vi "FindTemplateMethod.vi"(10 "TemplatePath To Use first":path, 11 "TemplatePath in":path) -> (3 "TemplatePath out":path)   [LabVIEW 2020, in "ClassWriterNative.lvclass"]
uses:
  ClassWriterNative.lvclass
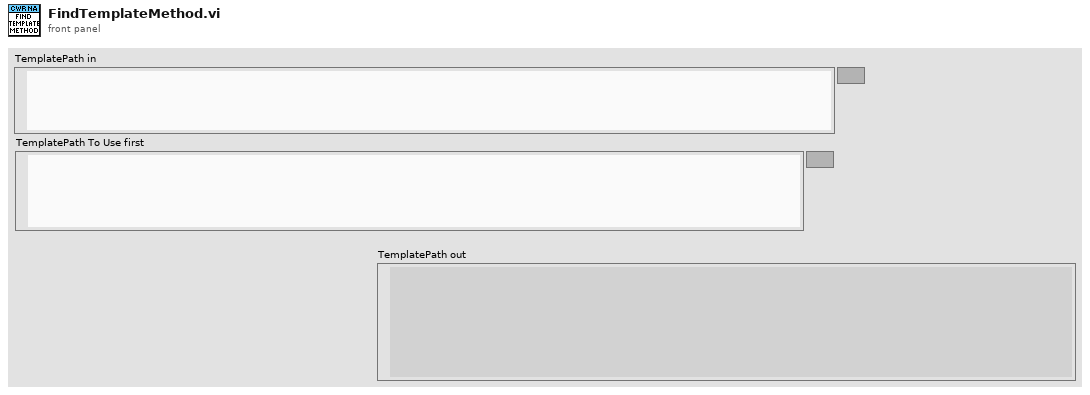
[diagram p1: front panel]
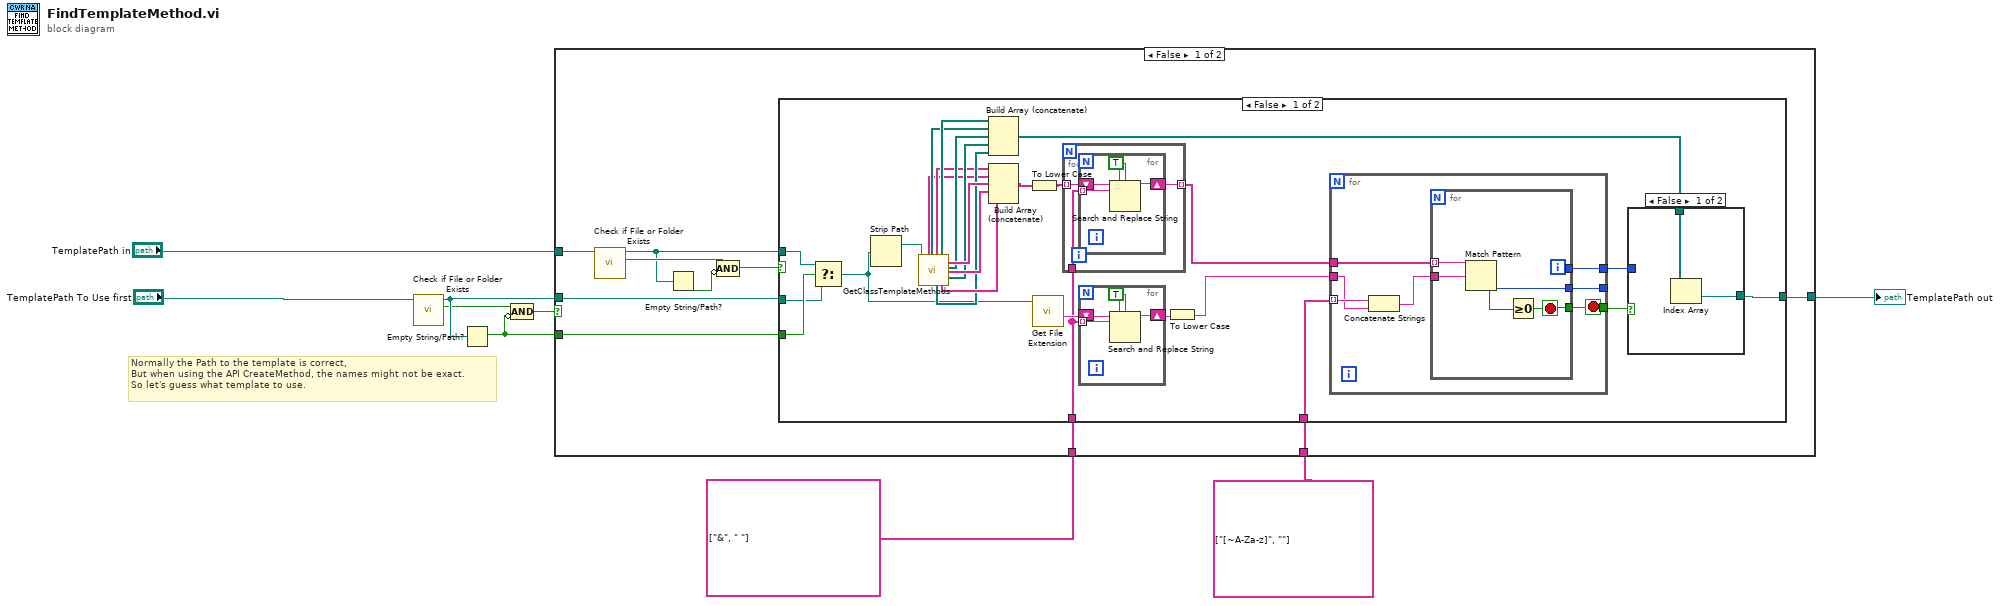
[diagram p0: block diagram]
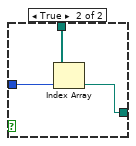
[diagram p2: hidden frame]
diagram:
  # "Normally the Path to the template is correct, \nBut when using the API CreateMethod, the names might not be exact.\nSo let's guess what template to use."
  n1 = call <vilib>:"Check if File or Folder Exists.vi"("path"="TemplatePath To Use first") -> ("file or folder exists?"=w5:bool, "dup path"=w6:path)  [unwired: 8 in, 1 out]
  n2 = Empty String/Path?(string/path=w6) -> (empty?=w1:bool)
  n3 = Compound Arithmetic op=AND(w5, invert w1) -> (w4:bool)
  n4 = case shown="False" w4 {
    tunnel: [w15 w76] -> w8
    tunnel: w6 -> [w12 w76]
    tunnel: "TemplatePath in" -> [w19 _]
    tunnel: string[] ["&", " "] -> [w14 _]
    tunnel: string[] ["[~A-Za-z]", ""] -> [w13 _]
    tunnel: w1 -> [w10 _]
    frame False {
      n5 = call <vilib>:"Check if File or Folder Exists.vi"("path"=w19) -> ("file or folder exists?"=w17:bool, "dup path"=w11:path)  [unwired: 8 in, 1 out]
      n6 = Empty String/Path?(string/path=w11) -> (empty?=w18:bool)
      n7 = Compound Arithmetic op=AND(w17, invert w18) -> (w16:bool)
      n8 = case shown="False" w16 {
        tunnel: w12 -> [w26 _]
        tunnel: [w30 w75] -> w15
        tunnel: w14 -> [w32 _]
        tunnel: w13 -> [w43 _]
        tunnel: w11 -> [w25 w75]
        tunnel: w10 -> [w27 _]
        frame False {
          n9 = Select(t=w25, s=w27, f=w26) -> (s? t:f=w24:path)
          n10 = Strip Path(path=w24) -> (stripped path=w28:path)  [unwired: 1 out]
          n11 = call "GetClassTemplateMethods.vi"("MethodTemplatePath"=w28) -> ("InterfaceMethodNames"=w20:string[], "InterfaceMethodPaths"=w22:path[], "NormalMethodNames"=w21:string[], "PropertyNodeMethodPaths"=w37:path[], "NormalMethodPaths"=w23:path[], "PropertyNodeMethodNames"=w40:string[], "OverrideMethodNames"=w42:string[], "OverrideMethodPaths"=w39:path[], "PropertyMethodNames"=w41:string[], "PropertyMethodPaths"=w38:path[])  [unwired: 8 in, 1 out]
          n12 = Build Array (concatenate)(w23, w22, w39, w38, w37) -> (w34:path[])
          n13 = Build Array (concatenate)(w21, w20, w42, w41, w40) -> (w36:string[])
          n14 = To Lower Case(string=w36) -> (all lower case string=w33:string[])
          n15 = call <vilib>:"Get File Extension.vi"("file"=w24) -> ("filename without extension"=w46:string)  [unwired: 6 in, 4 out]
          n16 = for {
            tunnel: w33 -> [w54] mode=indexing
            tunnel: w32 -> [w53]
            tunnel: [w52] -> w31 mode=indexing
            n17 = for {
              tunnel: w53 -> [w56] mode=indexing
              shift-right: [w55] -> w52
              shift-left: w54 -> [w58]
              w57 = TRUE ("replace all? (F)")
              n18 = Search and Replace String(replace all?=w57, case sensitive?=w57, input string=w58, search string=w56) -> (result string=w55:string)  [unwired: 4 in, 3 out]
            }
          }
          n19 = for {
            tunnel: w32 -> [w72] mode=indexing
            shift-right: [w71] -> w45
            shift-left: w46 -> [w74]
            w73 = TRUE ("replace all? (F)")
            n20 = Search and Replace String(replace all?=w73, case sensitive?=w73, input string=w74, search string=w72) -> (result string=w71:string)  [unwired: 4 in, 3 out]
          }
          n21 = To Lower Case(string=w45) -> (all lower case string=w44:string)
          n22 = for {
            tunnel: w31 -> [w65]
            tunnel: w44 -> [w63]
            tunnel: w43 -> [w64] mode=indexing
            tunnel: [w61] -> _
            tunnel: [w60] -> w35
            tunnel: [w59] -> w29
            stop <- w59 stop-if-true
            n23 = Concatenate Strings(w64, w63) -> (w62:string)
            n24 = for {
              tunnel: w65 -> [w70] mode=indexing
              tunnel: w62 -> [w69]
              tunnel: [w68] -> w59
              tunnel: [w67] -> w61
              tunnel: [w66] -> w60
              i -> [w66]
              stop <- w68 stop-if-true
              n25 = Match Pattern(string=w70, regular expression=w69) -> (offset past match=w67:i32)  [unwired: 1 in, 3 out]
              n26 = Greater Or Equal To 0?(x=w67) -> (x >= 0?=w68:bool)
            }
          }
          n27 = case shown="False" w29 {
            tunnel: w35 -> [_ w51]
            tunnel: w34 -> [w48 w50]
            tunnel: [w47 w49] -> w30
            frame False {
              n28 = Index Array(array=w48) -> (element=w47:path)  [unwired: 1 in]
            }
            frame True {
              n29 = Index Array(array=w50, index=w51) -> (element=w49:path)
            }
          }
        }
        frame True {
        }
      }
    }
    frame True {
    }
  }
  "TemplatePath out" <- w8
